vi "Set Message Metatdata.vi"(6 "Message Type":T1, 8 "error in (no error)":errorcluster, 10 "References":T2) -> (0 "error out":errorcluster)   [LabVIEW 2023, in "Message Maker.lvclass"]
doc: "Writes checksums and message info to the message class's meta data. These checksums are used to detect changes in the source VIs\n\nAuthor: Derek Trepanier\nCopyright: MGI 2015"
uses:
  Message Maker.lvclass
  Scripting Refs.ctl
  Message Type.ctl
  Method Signature.ctl
  <vilib>/LabVIEW Icon API/lv_icon/Classes/Icon/Icon.lvclass
  <vilib>/LabVIEW Icon API/LabVIEW Icon API.lvlib
panel:
  out "Array":string[](array[string])
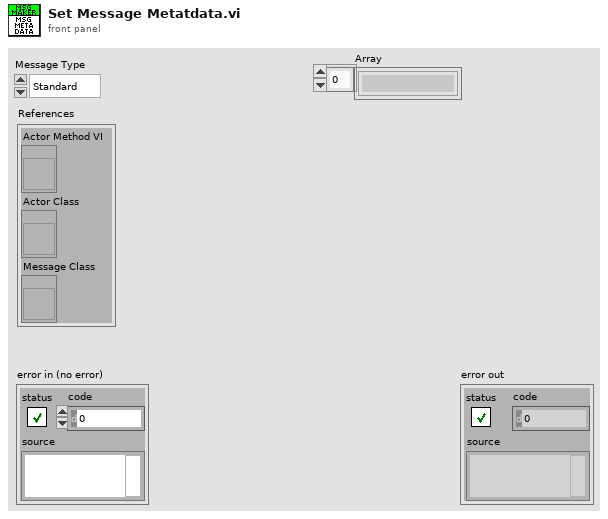
[diagram p1: front panel]
types:
  T1 = typedef "Message Maker.lvclass/Message Type.ctl" = enum16{"Standard", "Async"}
  T2 = typedef "Message Maker.lvclass/Scripting Refs.ctl" = cluster{"Actor Method VI":refnum<vi>, "Actor Class":refnum<vi>, "Message Class":refnum<vi>}
  T3 = typedef "Message Maker.lvclass/Method Signature.ctl" = cluster{"Connector Pane":variant, "Description":string, "Icon":refnum<class "Icon.lvclass">}
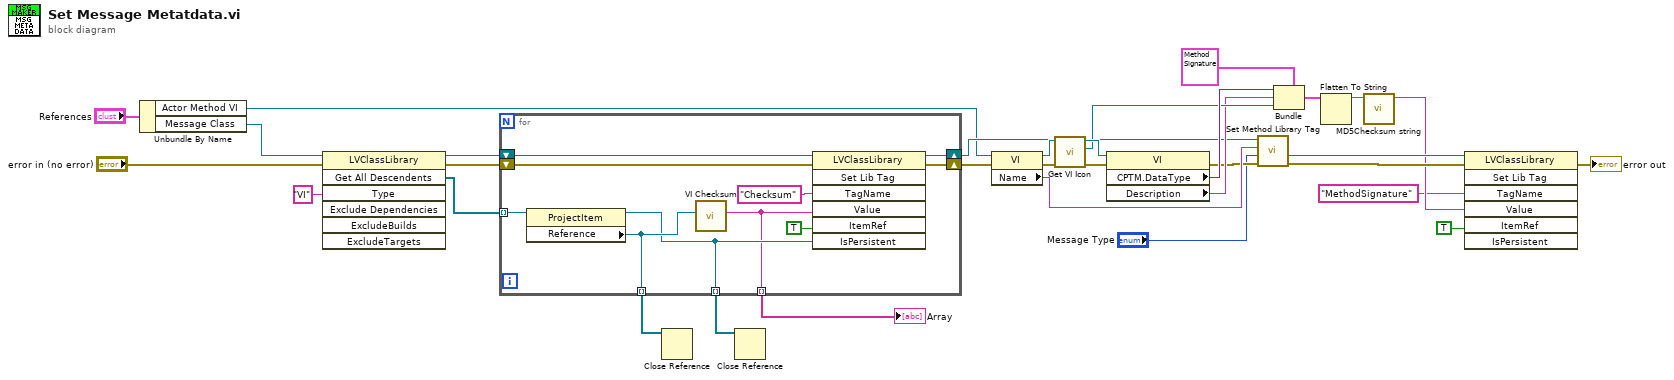
[diagram p0: block diagram]
diagram:
  n1 = Unbundle By Name("References") -> ("Actor Method VI"=w1:refnum<vi>, "Message Class"=w14:refnum<vi>)
  n2 = invoke class="LVClassLibrary" method="Get All Descendents"(reference=w14, error in="error in (no error)", "Type"="VI") -> (reference out=w10:refnum<vi>, error out=w9:errorcluster, "All Descendents"=w7:refnum<vi>[])  [unwired: 4 in, 4 out]
  n3 = for {
    tunnel: w7 -> [w42] mode=indexing
    shift-right: [w40] -> w13
    shift-left: w10 -> [w41]
    shift-right: [w38] -> w12
    shift-left: w9 -> [w39]
    tunnel: [w35] -> w5 mode=indexing
    tunnel: [w34] -> w6 mode=indexing
    tunnel: [w33] -> w4 mode=indexing
    n4 = property class="ProjectItem"(reference=w42) -> (reference out=w34:refnum<vi>, "Reference"=w35:refnum<vi>)  [unwired: 1 in, 1 out]
    n5 = call "VI Checksum.vi"("VI"=w35) -> ("VI Checksum"=w33:string)  [unwired: 10 in]
    n6 = invoke class="LVClassLibrary" method="Set Lib Tag"(reference=w41, error in=w39, "TagName"="Checksum" ("Tag Name"), "Value"=w33, "ItemRef"=TRUE ("Is Persistent"), "IsPersistent"=w34) -> (reference out=w40:refnum<vi>, error out=w38:errorcluster)  [unwired: 1 in, 5 out]
  }
  "Array" <- w4
  n7 = Close Reference(reference=w5) -> ()  [unwired: 1 in, 1 out]
  n8 = Close Reference(reference=w6) -> ()  [unwired: 1 in, 1 out]
  n9 = property class="VI"(reference=w1, error in=w12) -> (reference out=w27:refnum<vi>, error out=w25:errorcluster, "Name"=w26:string)
  n10 = call <vilib>:"Get VI Icon.vi"("error in (no error)"=w25, "VI Refnum in"=w27) -> ("error out"=w24:errorcluster, "Icon"=w30:refnum<class "Icon.lvclass">, "VI Refnum out"=w32:refnum<vi>)  [unwired: 7 in]
  n11 = property class="VI"(reference=w32, error in=w24) -> (error out=w23:errorcluster, "CPTM.DataType"=w31:variant, "Description"=w29:string)  [unwired: 1 out]
  n12 = call "Set Method Library Tag.vi"("error in (no error)"=w23, "Message Type"="Message Type", "VI FQN"=w26, "LVClassLibrary in"=w13) -> ("error out"=w20:errorcluster, "LVClassLibrary out"=w22:refnum<vi>)  [unwired: 6 in]
  n13 = Bundle(cluster=T3 {"Connector Pane"=variant, "Description"="", "Icon"=refnum} ("output cluster"), "Connector Pane"=w31, "Description"=w29, "Icon"=w30) -> (w17:T3)
  n14 = Flatten To String(anything=w17) -> (data string=w16:string)  [unwired: 3 in, 2 out]
  n15 = call <vilib>:"MD5Checksum string.vi"("Message String"=w16) -> ("MD5 message-digest"=w15:string)  [unwired: 10 in]
  n16 = invoke class="LVClassLibrary" method="Set Lib Tag"(reference=w22, error in=w20, "TagName"="MethodSignature" ("Tag Name"), "Value"=w15, "ItemRef"=TRUE ("Is Persistent")) -> (error out=→"error out":errorcluster)  [unwired: 2 in, 6 out]
